vi "Parse LTE Call Process Param.vi"(8 "error in (no error)":errorcluster caption="에러 입력(에러 없음)", 10 "JSON string":string, 11 "Instrument Manager 입력":refnum<class "Instrument Manager.lvclass">) -> (0 "error out":errorcluster caption="에러 출력", 1 "LTE Call Process Param":T1, 2 "Call Process Param LTE":T3, 3 "Instrument Manager 출력":refnum<class "Instrument Manager.lvclass">)   [LabVIEW 2023, in "Instrument Manager.lvclass"]
uses:
  Instrument Manager.lvclass
  Call Process Param LTE.ctl
  Type Definition/LTE Call Process Param.ctl
  Module/ANRITSU Call Box/Type Definition/LTE Supported BandWidth.ctl
  Instrument Manager.lvclass/Instrument Manager.ctl
  Module/ANRITSU Call Box/ANRITSU Call Box.lvlib
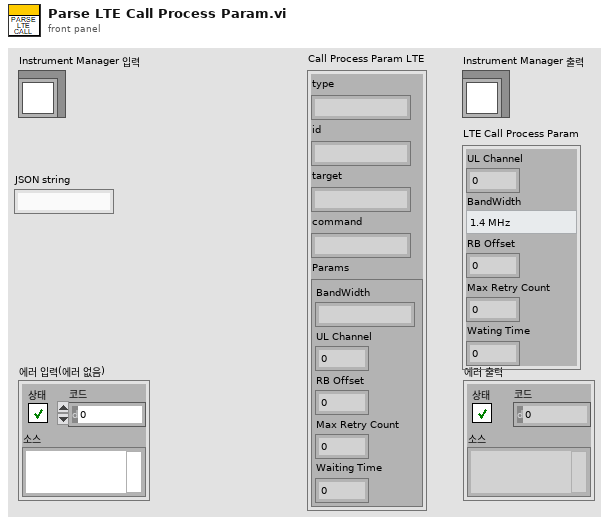
[diagram p1: front panel]
types:
  T1 = typedef "LTE Call Process Param.ctl" = cluster{"UL Channel":i32, "BandWidth":T2, "RB Offset":i32, "Max Retry Count":i32, "Wating Time":i32}
  T2 = typedef "ANRITSU Call Box.lvlib/LTE Supported BandWidth.ctl" = enum16{"1.4 MHz", "3 MHz", "5 MHz", "10 MHz", "15 MHz", "20 MHz"}
  T3 = typedef "Instrument Manager.lvclass/Call Process Param LTE.ctl" = cluster{"type":string, "id":string, "target":string, "command":string, "Params":cluster{"BandWidth":string, "UL Channel":i32, "RB Offset":i32, "Max Retry Count":i32, "Waiting Time":i32}}
  T4 = cluster{"BandWidth":string, "UL Channel":i32, "RB Offset":i32, "Max Retry Count":i32, "Waiting Time":i32}
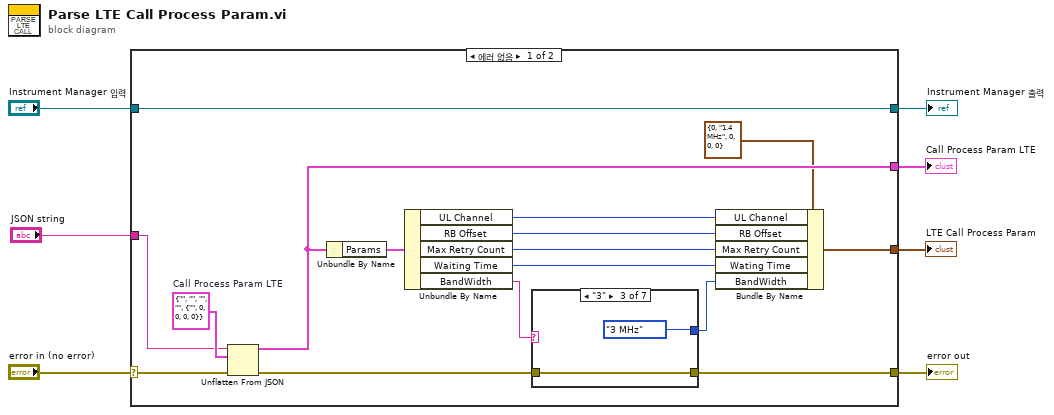
[diagram p0: block diagram]
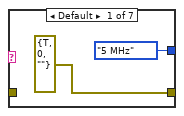
[diagram p2: hidden frame]
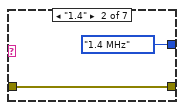
[diagram p3: hidden frame]
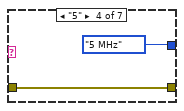
[diagram p4: hidden frame]
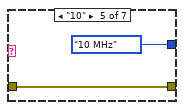
[diagram p5: hidden frame]
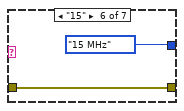
[diagram p6: hidden frame]
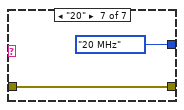
[diagram p7: hidden frame]
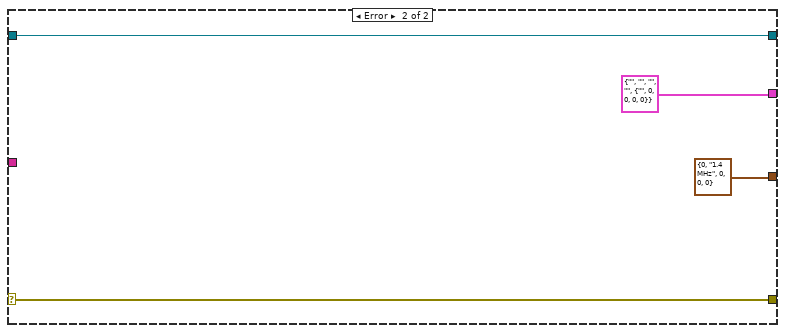
[diagram p8: hidden frame]
diagram:
  n1 = case shown="에러 없음" "error in (no error)" {
    selector: "error in (no error)" -> [w22 w41]
    tunnel: [w14 w41] -> w6
    tunnel: [w23 w40] -> w4
    tunnel: "Instrument Manager 입력" -> [w23 w40]
    tunnel: "JSON string" -> [w20 _]
    tunnel: [w19 T3 {"type"="", "id"="", "target"="", "command"="", "Params"={"BandWidth"="", "UL Channel"=0, "RB Offset"=0, "Max Retry Count"=0, "Waiting Time"=0}} ("Call Process Param LTE")] -> w2
    tunnel: [w8 T1 {"UL Channel"=0, "BandWidth"=enum."1.4 MHz", "RB Offset"=0, "Max Retry Count"=0, "Wating Time"=0} ("LTE Call Process Param")] -> w1
    frame No Error {
      w21 = T3 {"type"="", "id"="", "target"="", "command"="", "Params"={"BandWidth"="", "UL Channel"=0, "RB Offset"=0, "Max Retry Count"=0, "Waiting Time"=0}}  # Call Process Param LTE
      n2 = Unflatten From JSON(JSON string=w20, type and defaults=w21, error in (no error)=w22) -> (value=w19:T3, error out=w16:errorcluster)  [unwired: 4 in]
      n3 = Unbundle By Name(w19) -> ("Params"=w18:T4)
      n4 = Unbundle By Name(w18) -> ("UL Channel"=w12:i32, "RB Offset"=w11:i32, "Max Retry Count"=w10:i32, "Waiting Time"=w9:i32, "BandWidth"=w17:string)
      n5 = case shown="\"3\"" w17 {
        tunnel: w16 -> [_ w27 w29 w31 w32 w34 w36]
        tunnel: [errorcluster {"status"=TRUE, "code"=0, "source"=""} ("error out") w27 w29 w31 w32 w34 w36] -> w14
        tunnel: [LTE_Supported_BandWidth."5 MHz" ("BandWidth") LTE_Supported_BandWidth."1.4 MHz" ("BandWidth") LTE_Supported_BandWidth."3 MHz" ("BandWidth") LTE_Supported_BandWidth."5 MHz" ("BandWidth") LTE_Supported_BandWidth."10 MHz" ("BandWidth") LTE_Supported_BandWidth."15 MHz" ("BandWidth") LTE_Supported_BandWidth."20 MHz" ("BandWidth")] -> w13
        frame Default {
        }
        frame "1.4" {
        }
        frame "3" {
        }
        frame "5" {
        }
        frame "10" {
        }
        frame "15" {
        }
        frame "20" {
        }
      }
      n6 = Bundle By Name(cluster=T1 {"UL Channel"=0, "BandWidth"=enum."1.4 MHz", "RB Offset"=0, "Max Retry Count"=0, "Wating Time"=0} ("LTE Call Process Param"), "UL Channel"=w12, "RB Offset"=w11, "Max Retry Count"=w10, "Wating Time"=w9, "BandWidth"=w13) -> (w8:T1)
    }
    frame Error {
    }
  }
  "error out" <- w6
  "Instrument Manager 출력" <- w4
  "Call Process Param LTE" <- w2
  "LTE Call Process Param" <- w1
